vi "DQMH_API_CleanUp.vi"(11 "error in (no error)":errorcluster) -> (15 "error out":errorcluster)   [LabVIEW 2020, in "DQMH_API.lvclass"]
uses:
  <resource>/Framework/Providers/Open_GDS/UML/DQMH_API_class/DQMH_API.lvclass
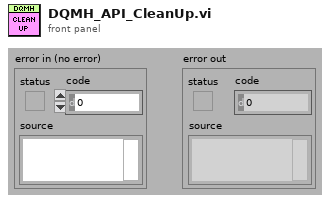
[diagram p1: front panel]
types:
  T1 = typedef "DQMH_API.lvclass/ObjectAttributes.ctl" = cluster{"Get Module Type Info":refnum<vi>, "Script New Module":refnum<vi>, "Script New Event":refnum<vi>, "Query Library for Module Info":refnum<vi>, "Parse Project for DQMH Modules":refnum<vi>, "Get All Events in Module":refnum<vi>}
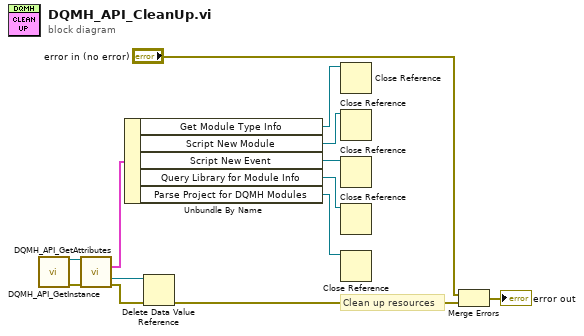
[diagram p0: block diagram]
diagram:
  # "Clean up resources"
  n1 = call <resource>:"DQMH_API_GetInstance.vi"() -> ("reference out"=w10:refnum<class "DQMH_API.lvclass">, "error out"=w11:errorcluster)  [unwired: 11 in, 3 out]
  n2 = call <resource>:"DQMH_API_GetAttributes.vi"("reference in"=w10, "error in (no error)"=w11) -> ("Data"=w12:T1, "DataRef"=w8:refnum<data-value>, "error out"=w9:errorcluster)  [unwired: 10 in, 1 out]
  n3 = Unbundle By Name(w12) -> ("Get Module Type Info"=w5:refnum<vi>, "Script New Module"=w4:refnum<vi>, "Script New Event"=w3:refnum<vi>, "Query Library for Module Info"=w2:refnum<vi>, "Parse Project for DQMH Modules"=w1:refnum<vi>)
  n4 = Delete Data Value Reference(data value reference=w8, error in=w9) -> (error out=w6:errorcluster)  [unwired: 1 out]
  n5 = Close Reference(reference=w5) -> ()  [unwired: 1 in, 1 out]
  n6 = Close Reference(reference=w4) -> ()  [unwired: 1 in, 1 out]
  n7 = Close Reference(reference=w3) -> ()  [unwired: 1 in, 1 out]
  n8 = Close Reference(reference=w2) -> ()  [unwired: 1 in, 1 out]
  n9 = Close Reference(reference=w1) -> ()  [unwired: 1 in, 1 out]
  n10 = Merge Errors("error in (no error)", w6) -> (→"error out":errorcluster)
